vi "Line Configuration Dialog.vi"(8 "error in":errorcluster, 9 "engine configuration in":refnum<class "engine configuration.lvclass">, 10 "tag bus configurable plugin module configuration":refnum<class "PID Module configuration.lvclass">, 11 "Line":T2) -> (0 "error out":errorcluster, 1 "success":bool, 2 "changed":bool, 3 "Mappings out":T1)   [LabVIEW 2015, in "PID Module editor node.lvclass"]
doc: "A dialog for allowing a user to specify the values of a new line."
uses:
  PID Module editor node.lvclass
  module/configuration/Line.ctl
  <vilib>/NI/Tag Bus Module Framework/channel/TBM channel.lvclass
  Mappings.ctl
  Map.ctl
  <vilib>/NI/Module Execution Interface/Engine Configuration/engine configuration.lvclass
  module/configuration/PID Module configuration.lvclass
  <vilib>/NI/Configuration Framework/serializable configuration/NISE_CEF_serializable configuration.lvclass/NISE_CEF_serializable configuration.ctl
  <vilib>/NI/Tag Bus/tag/tag descriptor.lvclass/tag descriptor.ctl
  <vilib>/NI/Tag Bus/tag/write tag name.vi
  <vilib>/NI/Configuration Framework/serializable configuration/Read UID.vi
  <vilib>/Utility/LVClass/Get LV Class Name.vi
  <vilib>/NI/Configuration Framework/error generator/NISE_error generator.vi
  <vilib>/NI/Tag Bus/tag/tag descriptor.lvclass
  <vilib>/NI/DCAF UI Toolkit/Controls/DCAF UI Elements.lvlib
panel:
  out "errors":string
  in  "Tag":i32(listbox)
  in  "PID Id":string
  in  "cancel":bool
  in  "ok":bool
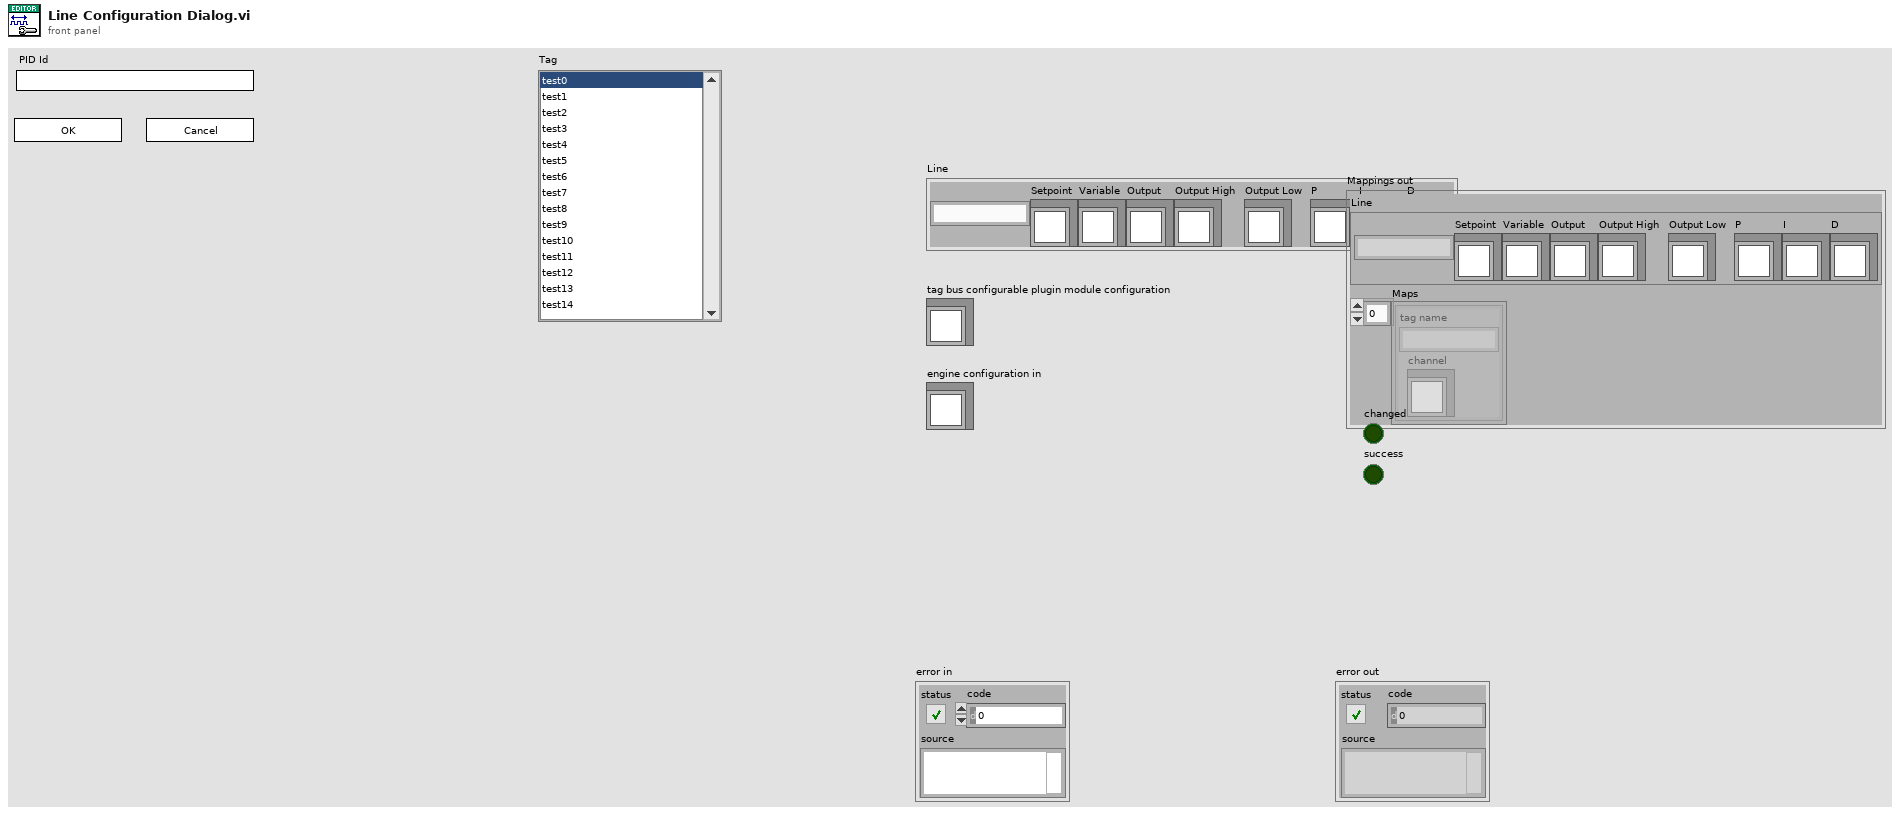
[diagram p1: front panel]
types:
  T1 = typedef "PID Module editor node.lvclass/Mappings.ctl" = cluster{"Line":T2, "Maps":T3[]}
  T2 = typedef "PID Module configuration.lvclass/Line.ctl" = cluster{"PID ID":string, "Setpoint":refnum<class "TBM channel.lvclass">, "Variable":refnum<class "TBM channel.lvclass">, "Output":refnum<class "TBM channel.lvclass">, "Output High":refnum<class "TBM channel.lvclass">, "Output Low":refnum<class "TBM channel.lvclass">, "P":refnum<class "TBM channel.lvclass">, "I":refnum<class "TBM channel.lvclass">, "D":refnum<class "TBM channel.lvclass">}
  T3 = typedef "PID Module editor node.lvclass/Map.ctl" = cluster{"channel":refnum<class "TBM channel.lvclass">, "tag name":string}
  T4 = enum8{"Enabled", "Disabled", "Disabled and Grayed Out"}
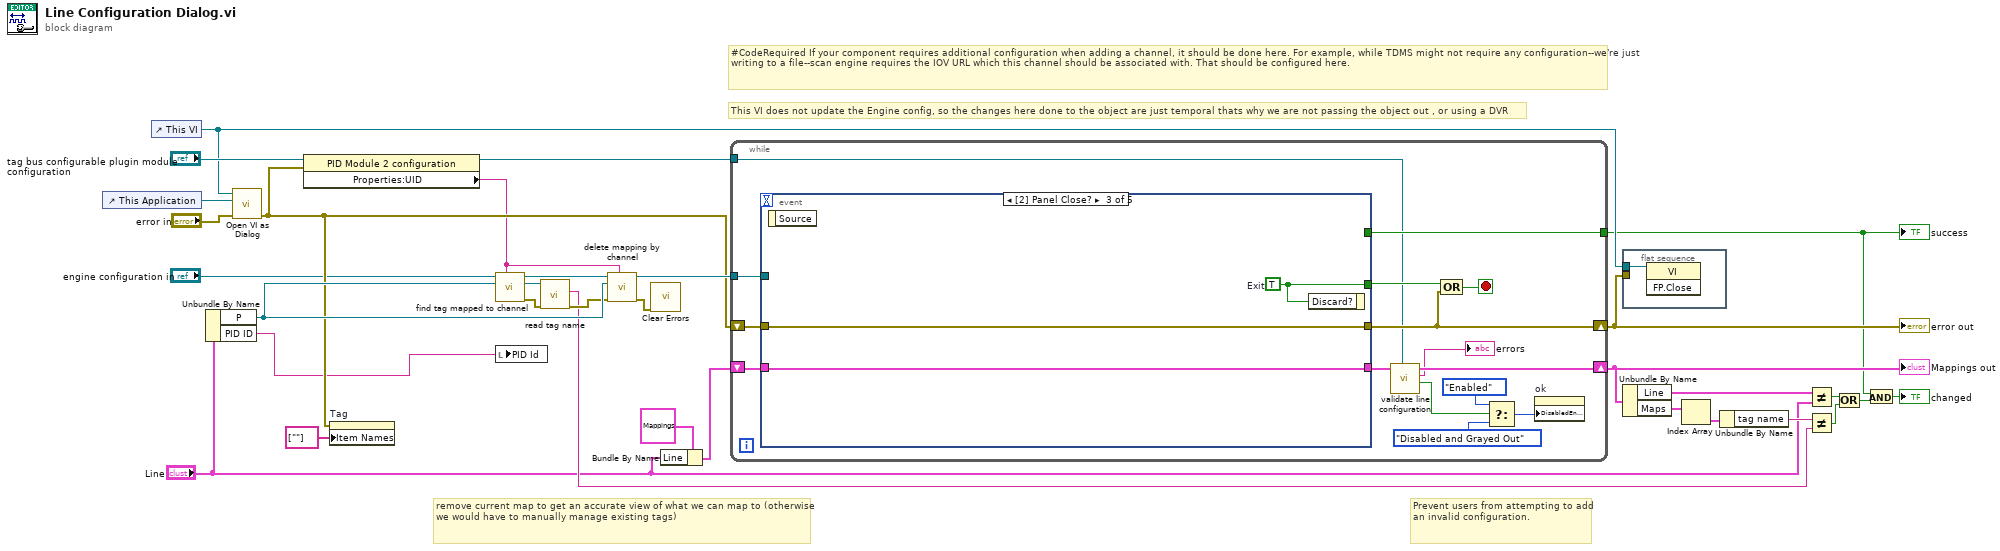
[diagram p0: block diagram]
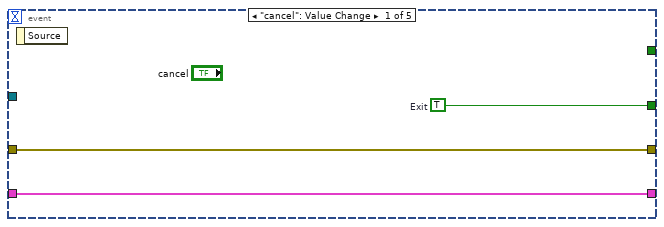
[diagram p2: hidden frame]
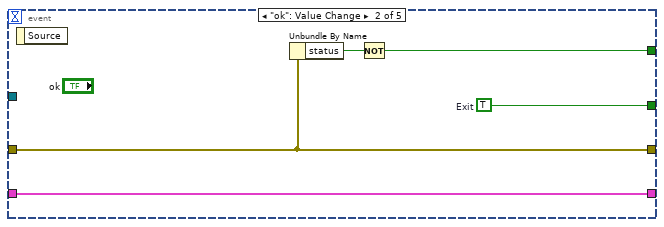
[diagram p3: hidden frame]
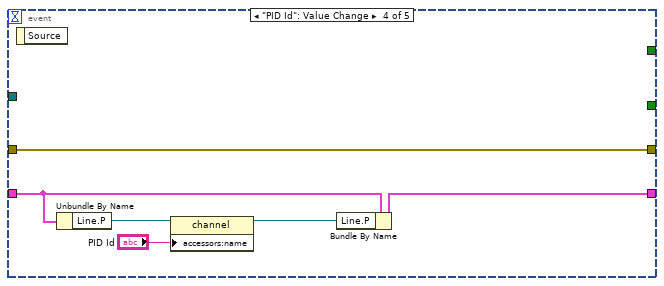
[diagram p4: hidden frame]
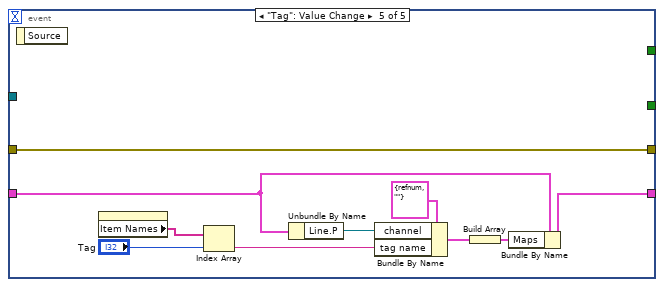
[diagram p5: hidden frame]
diagram:
  # "Prevent users from attempting to add an invalid configuration."
  # "This VI does not update the Engine config, so the changes here done to the object are just temporal thats why we are not passing the object out , or using a DVR"
  # "remove current map to get an accurate view of what we can map to (otherwise we would have to manually manage existing tags)"
  # "#CodeRequired If your component requires additional configuration when adding a channel, it should be done here. For example, while TDMS might not require any configuration--we're just writing to a file--scan engine requires the IOV URL which this channel should be associated with. That should be configured here."
  n1 = control-ref of="This Application"() -> (w23:refnum<vi>)
  n2 = control-ref of="This VI"() -> (w9:refnum<vi>)
  n3 = Unbundle By Name("Line") -> ("P"=w31:refnum<class "TBM channel.lvclass">, "PID ID"=w1:string)
  n4 = call <vilib>:"Open VI as Dialog.vi"("error in (no error)"="error in", "This Application"=w23, "VI in"=w9) -> ("error out"=w21:errorcluster)  [unwired: 8 in]
  n5 = property class="PID Module 2 configuration"(reference="tag bus configurable plugin module configuration", error in=w21) -> (reference out=w18:refnum<class "PID Module configuration.lvclass">, "Properties:UID"=w6:string)  [unwired: 1 out]
  n6 = property on="Tag" class="LstBox (strict)"(error in=w21, "Item Names"=string[] [""]) -> ()  [unwired: 1 in, 2 out]
  n7 = call <vilib>:"find tag mapped to channel.vi"("owner"=w6, "channel"=w31, "engine configuration in"="engine configuration in") -> ("error out"=w16:errorcluster, "tag"=w17:refnum<class "tag descriptor.lvclass">, "engine configuration out"=w19:refnum<class "engine configuration.lvclass">)  [unwired: 6 in]
  n8 = local write "PID Id"(w1) -> ()
  n9 = call <vilib>:"read tag name.vi"("error in"=w16, "system tag in"=w17) -> ("error out"=w15:errorcluster, "name"=w8:string)  [unwired: 7 in, 1 out]
  n10 = call <vilib>:"delete mapping by channel.vi"("owner ID"=w6, "error in"=w15, "channel"=w31, "engine configuration in"=w19) -> ("error out"=w29:errorcluster, "engine configuration out"=w32:refnum<class "engine configuration.lvclass">)  [unwired: 6 in]
  n11 = call <vilib>:"Clear Errors.vi"("error in (no error)"=w29) -> ()  [unwired: 5 in, 2 out]
  n12 = Bundle By Name(cluster=T1 {"Line"={"PID ID"="", "Setpoint"=refnum, "Variable"=refnum, "Output"=refnum, "Output High"=refnum, "Output Low"=refnum, "P"=refnum, "I"=refnum, "D"=refnum}, "Maps"=[]} ("Mappings out"), "Line"="Line") -> (w26:T1)
  n13 = while {
    shift-right: [w39] -> w5
    shift-left: w21 -> [w46]
    tunnel: [w45] -> w4
    shift-right: [w40] -> w24
    shift-left: w26 -> [w42]
    tunnel: w32 -> [w47]
    tunnel: w18 -> [w34]
    stop <- w43 stop-if-true
    n14 = event shown="[2] Panel Close?" {
      selector: _ -> [_ _ _ _ _]
      dyn-events: _ -> [_ _ _ _ _]
      timeout: _ -> [_ _ _ _ _]
      tunnel: w47 -> [_ _ _ _ _]
      tunnel: w46 -> [w50 w53 w58 w64 w74]
      tunnel: [w50 w53 w58 w64 w74] -> w39
      tunnel: [_ w51 _ _ _] -> w45
      tunnel: [w48 w54 w56 _ _] -> w44
      tunnel: w42 -> [w49 w55 w57 w62 w65]
      tunnel: [w49 w55 w57 w63 w67] -> w41
      event "cancel": Value Change {
        w48 = TRUE  # Exit
        n15 = event-data() -> ()  [unwired: 1 in, 1 out]
      }
      event "ok": Value Change {
        w54 = TRUE  # Exit
        n16 = event-data() -> ()  [unwired: 1 in, 1 out]
        n17 = Unbundle By Name(w53) -> ("status"=w52:bool)
        n18 = Not(x=w52) -> (.not. x?=w51:bool)
      }
      event Panel Close? {
        w56 = TRUE  # Exit
        n19 = event-data() -> ()  [unwired: 1 in, 1 out]
        n20 = event-data("Discard?"=w56) -> ()  [unwired: 1 in, 1 out]
      }
      event "PID Id": Value Change {
        n21 = event-data() -> ()  [unwired: 1 in, 1 out]
        n22 = Unbundle By Name(w62) -> ("Line.P"=w61:refnum<class "TBM channel.lvclass">)
        n23 = property class="channel"(reference=w61, "accessors:name"="PID Id") -> (reference out=w60:refnum<class "TBM channel.lvclass">)  [unwired: 1 in, 1 out]
        n24 = Bundle By Name(cluster=w62, "Line.P"=w60) -> (w63:T1)
      }
      event "Tag": Value Change {
        n25 = event-data() -> ()  [unwired: 1 in, 1 out]
        n26 = property on="Tag" class="LstBox (strict)"() -> ("Item Names"=w72:string[])  [unwired: 2 in, 2 out]
        n27 = Index Array(array=w72, index="Tag") -> (element=w66:string)
        n28 = Unbundle By Name(w65) -> ("Line.P"=w70:refnum<class "TBM channel.lvclass">)
        n29 = Bundle By Name(cluster=T3 {"channel"=refnum, "tag name"=""} ("Map"), "channel"=w70, "tag name"=w66) -> (w69:T3)
        n30 = Build Array(w69) -> (w68:T3[])
        n31 = Bundle By Name(cluster=w65, "Maps"=w68) -> (w67:T1)
      }
    }
    n32 = call "validate line configuration.vi"("Module Config"=w34, "Mappings in"=w41) -> ("valid?"=w38:bool, "errors"=→"errors":string, "Mappings out"=w40:T1)  [unwired: 7 in]
    n33 = Compound Arithmetic op=OR(w44, w39) -> (w43:bool)
    n34 = Select(t=T4."Enabled" ("Disabled"), s=w38, f=T4."Disabled and Grayed Out") -> (s? t:f=w35:T4)
    n35 = property on="ok" class="Bool"("DisabledEnum"=w35) -> ()  [unwired: 2 in, 2 out]
  }
  "error out" <- w5
  "success" <- w4
  "Mappings out" <- w24
  n36 = flat-sequence {
    tunnel: w5 -> [_]
    tunnel: w9 -> [w75]
    frame #0 {
      n37 = invoke class="VI" method="FP.Close"(reference=w75) -> ()  [unwired: 2 in, 3 out]
    }
  }
  n38 = Unbundle By Name(w24) -> ("Line"=w25:T2, "Maps"=w14:T3[])
  n39 = Index Array(array=w14) -> (element=w13:T3)  [unwired: 1 in]
  n40 = Unbundle By Name(w13) -> ("tag name"=w12:string)
  n41 = Not Equal?(x=w25, y="Line") -> (x != y?=w10:bool)
  n42 = Not Equal?(x=w12, y=w8) -> (x != y?=w11:bool)
  n43 = Or(x=w10, y=w11) -> (x .or. y?=w3:bool)
  n44 = And(x=w4, y=w3) -> (x .and. y?=→"changed":bool)
